vi "beep_detection_2.vi"() -> (2 "Beep":bool)   [LabVIEW 2026]
uses:
  <vilib>/sound2/lvsound2.llb/Sampling Mode.ctl
  <vilib>/sound2/lvsound2.llb/Sound Data Format.ctl
  <vilib>/sound2/lvsound2.llb/Sound File Refnum.ctl
  <vilib>/sound2/lvsound2.llb/Sound File Write Open.vi
  <vilib>/sound2/lvsound2.llb/Sound Input Read (DBL).vi
  <vilib>/sound2/lvsound2.llb/Sound File Write (DBL).vi
panel:
  in  "Write Test File":bool
  in  "file path":path=path "C:/Users/Public/test.wav"
  in  "Volume Threshold":dbl=0.085
  out "max":dbl
  in  "sound format 3":T1={"sample rate (S/s)"=16000.0, "number of channels"=1, "bits per sample"=8}
  in  "number of samples/ch 3":i32=1000
  in  "sample mode 3":T2=1 items=["Finite Samples", "Continuous Samples"]
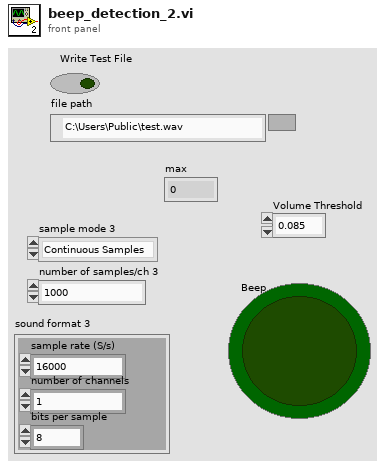
[diagram p1: front panel]
types:
  T1 = typedef "Sound Data Format.ctl" = cluster{"sample rate (S/s)":dbl, "number of channels":i32, "bits per sample":i32}
  T2 = typedef "Sampling Mode.ctl" = i32
  T3 = typedef "Sound Input Task ID.ctl" = u32
  T4 = typedef "Sound File Refnum.ctl" = refnum<file>
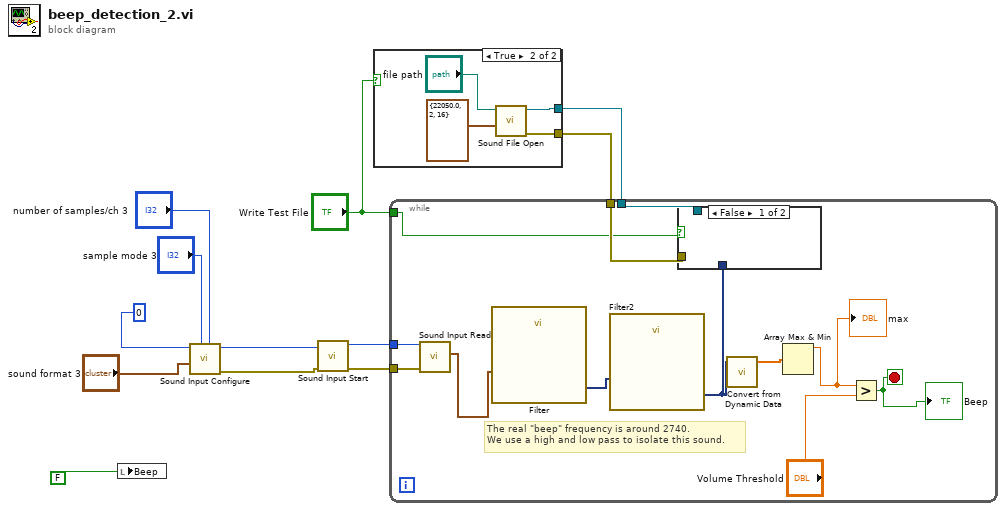
[diagram p0: block diagram]
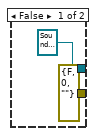
[diagram p2: hidden frame]
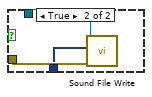
[diagram p3: hidden frame]
diagram:
  n1 = local write "Beep"(FALSE ("Beep")) -> ()
  n2 = call <vilib>:"Sound Input Configure.vi"("number of samples/ch"="number of samples/ch 3", "sample mode"="sample mode 3", "sound format"="sound format 3", "device ID"=u32 0) -> ("error out"=w10:errorcluster, "task ID"=w9:T3)  [unwired: 6 in]
  n3 = call <vilib>:"Sound Input Start.vi"("error in (no error)"=w10, "task ID"=w9) -> ("error out"=w7:errorcluster, "task ID out"=w6:T3)  [unwired: 8 in]
  n4 = case shown="True" "Write Test File" {
    tunnel: [T4 refnum ("sound file refnum") w18] -> w4
    tunnel: [errorcluster {"status"=FALSE, "code"=0, "source"=""} ("error out") w16] -> w3
    frame False {
    }
    frame True {
      n5 = call-poly <vilib>:"Sound File Open.vi"("sound format"=T1 {"sample rate (S/s)"=22050.0, "number of channels"=2, "bits per sample"=16}, "path"="file path") -> ("error out"=w16:errorcluster, "sound file refnum"=w18:T4)  [unwired: 8 in]
    }
  }
  n6 = while {
    tunnel: w7 -> [w30]
    tunnel: w6 -> [w29]
    tunnel: w4 -> [w28]
    tunnel: w3 -> [w27]
    tunnel: "Write Test File" -> [w19]
    stop <- w22 stop-if-true
    # "The real \"beep\" frequency is around 2740.\nWe use a high and low pass to isolate this sound."
    n7 = call-poly <vilib>:"Sound Input Read.vi"("error in (no error)"=w30, "task ID"=w29) -> ("data"=w26:waveform(dbl)[])  [unwired: 7 in, 2 out]
    n8 = call "Filter"("Signal"=w26) -> ("Filtered Signal"=w25:dynamicdata)  [unwired: 9 in, 1 out]
    n9 = call "Filter2"("Signal"=w25) -> ("Filtered Signal"=w20:dynamicdata)  [unwired: 9 in, 1 out]
    n10 = case shown="False" w19 {
      tunnel: w28 -> [_ w33]
      tunnel: w27 -> [_ w32]
      tunnel: w20 -> [_ w31]
      frame False {
      }
      frame True {
        n11 = call-poly <vilib>:"Sound File Write.vi"("error in (no error)"=w32, "data"=w31, "sound file refnum"=w33) -> ()  [unwired: 7 in, 2 out]
      }
    }
    n12 = call "Convert from Dynamic Data"("Dynamic Data Type"=w20) -> ("Array"=w24:dbl[])  [unwired: 3 in]
    n13 = Array Max & Min(array=w24) -> (max value=w23:dbl)  [unwired: 3 out]
    "max" <- w23
    n14 = Greater?(x=w23, y="Volume Threshold") -> (0:w22:bool)
    "Beep" <- w22
  }
